vi "TCP_Axis_Control(SubVI).vi"(0 "Speed Max":dbl, 1 "Step/s":dbl, 2 "Speed Mini":dbl, 3 "Position Max":dbl, 4 "User Input":dbl, 5 "Position Mini":dbl, 6 "Jog":sgl, 8 "Step/s Ref":refnum<vi>, 10 "User Input Ref":refnum<vi>, 12 "Moving Ref":refnum<vi>, 14 "Real Output Ref":refnum<vi>) -> (20 "Moving":bool, 22 "Real Output":dbl, 24 "TCP Forward":bool, 26 "TCP Backward":bool)   [LabVIEW 2018]
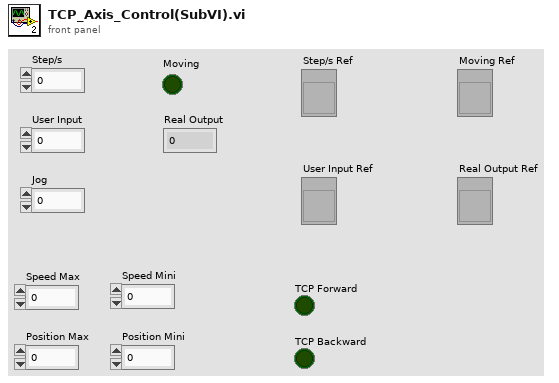
[diagram p1: front panel]
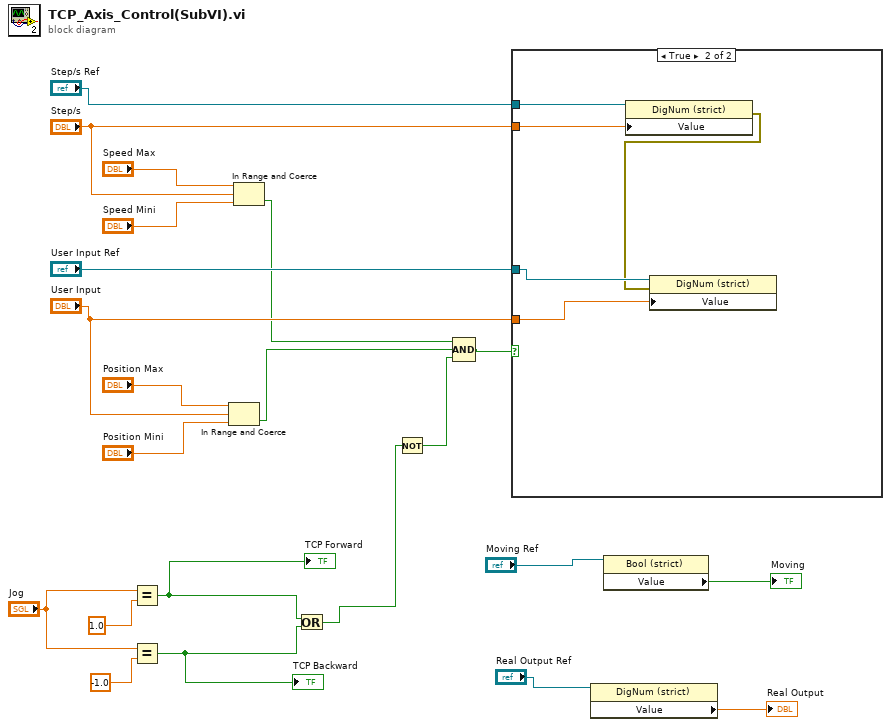
[diagram p0: block diagram]
diagram:
  n1 = Equal?(x="Jog", y=sgl 1.0) -> (x = y?=w4:bool)
  "TCP Forward" <- w4
  n2 = Equal?(x="Jog", y=sgl -1.0) -> (x = y?=w3:bool)
  "TCP Backward" <- w3
  n3 = In Range and Coerce(upper limit="Position Max", x="User Input", lower limit="Position Mini") -> (In Range?=w5:bool)  [unwired: 1 out]
  n4 = In Range and Coerce(upper limit="Speed Max", x="Step/s", lower limit="Speed Mini") -> (In Range?=w6:bool)  [unwired: 1 out]
  n5 = Or(x=w4, y=w3) -> (x .or. y?=w2:bool)
  n6 = Not(x=w2) -> (.not. x?=w1:bool)
  n7 = Compound Arithmetic op=AND(w6, w5, w1) -> (w7:bool)
  n8 = case shown="True" w7 {
    tunnel: "Step/s Ref" -> [_ w27]
    tunnel: "Step/s" -> [_ w26]
    tunnel: "User Input Ref" -> [_ w25]
    tunnel: "User Input" -> [_ w23]
    frame False {
    }
    frame True {
      n9 = property class="DigNum (strict)"(reference=w27, "Value"=w26) -> (error out=w24:errorcluster)  [unwired: 1 in, 1 out]
      n10 = property class="DigNum (strict)"(reference=w25, error in=w24, "Value"=w23) -> ()  [unwired: 2 out]
    }
  }
  n11 = property class="DigNum (strict)"(reference="Real Output Ref") -> ("Value"=→"Real Output":dbl)  [unwired: 1 in, 2 out]
  n12 = property class="Bool (strict)"(reference="Moving Ref") -> ("Value"=→"Moving":bool)  [unwired: 1 in, 2 out]
